vi "MQTT Packet - Send.vi"(0 "mqtt ref in":T1, 7 "packet data":u8[](array[numeric]), 9 "MessageType":T3, 11 "error in (no error)":errorcluster, 12 "Retain":bool, 13 "QoS":T2, 14 "DUP":bool) -> (3 "Debug":string, 4 "mqtt ref out":T1, 15 "error out":errorcluster)   [LabVIEW 2019, in "KoRE-MQTT.lvlib"]
doc: "Copyright (c) 2025 KoRElibs.com\nSPDX-License-Identifier: EUPL-1.2\n\nThis VI is licensed under the European Union Public License (EUPL) Version 1.2. You may use this VI unmodified in proprietary works. If you distribute a modified version of this file, the modified file must be released under the EUPL-1.2. Full license: https://joinup.ec.europa.eu/asset/eupl/eupl/1.2/"
uses:
  KoRE-MQTT.lvlib
  TypeDefs/MQTT Packet - Type.ctl
  Public/TypeDefs/MQTT QoS Level.ctl
  Public/TypeDefs/MQTT Client Session.ctl
  MQTT Data - Encode Varint.vi
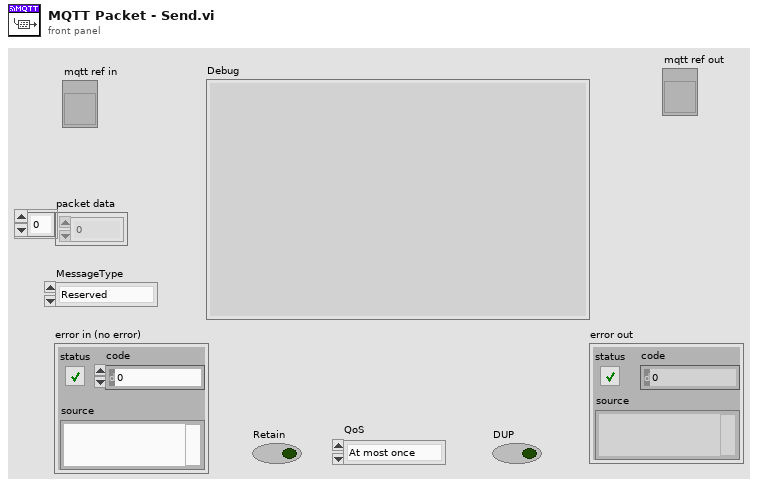
[diagram p1: front panel]
types:
  T1 = typedef "KoRE-MQTT.lvlib/MQTT Client Session.ctl" = refnum<vi>
  T2 = typedef "KoRE-MQTT.lvlib/MQTT QoS Level.ctl" = enum8{"At most once", "At least once", "Exactly once"}
  T3 = typedef "KoRE-MQTT.lvlib/MQTT Packet - Type.ctl" = enum32{"Reserved", "CONNECT", "CONNACK", "PUBLISH", "PUBACK", "PUBREC", "PUBREL", "PUBCOMP", "SUBSCRIBE", "SUBACK", "UNSUBSCRIBE", "UNSUBACK", "PINGREQ", "PINGRESP", "DISCONNECT", "AUTH"}
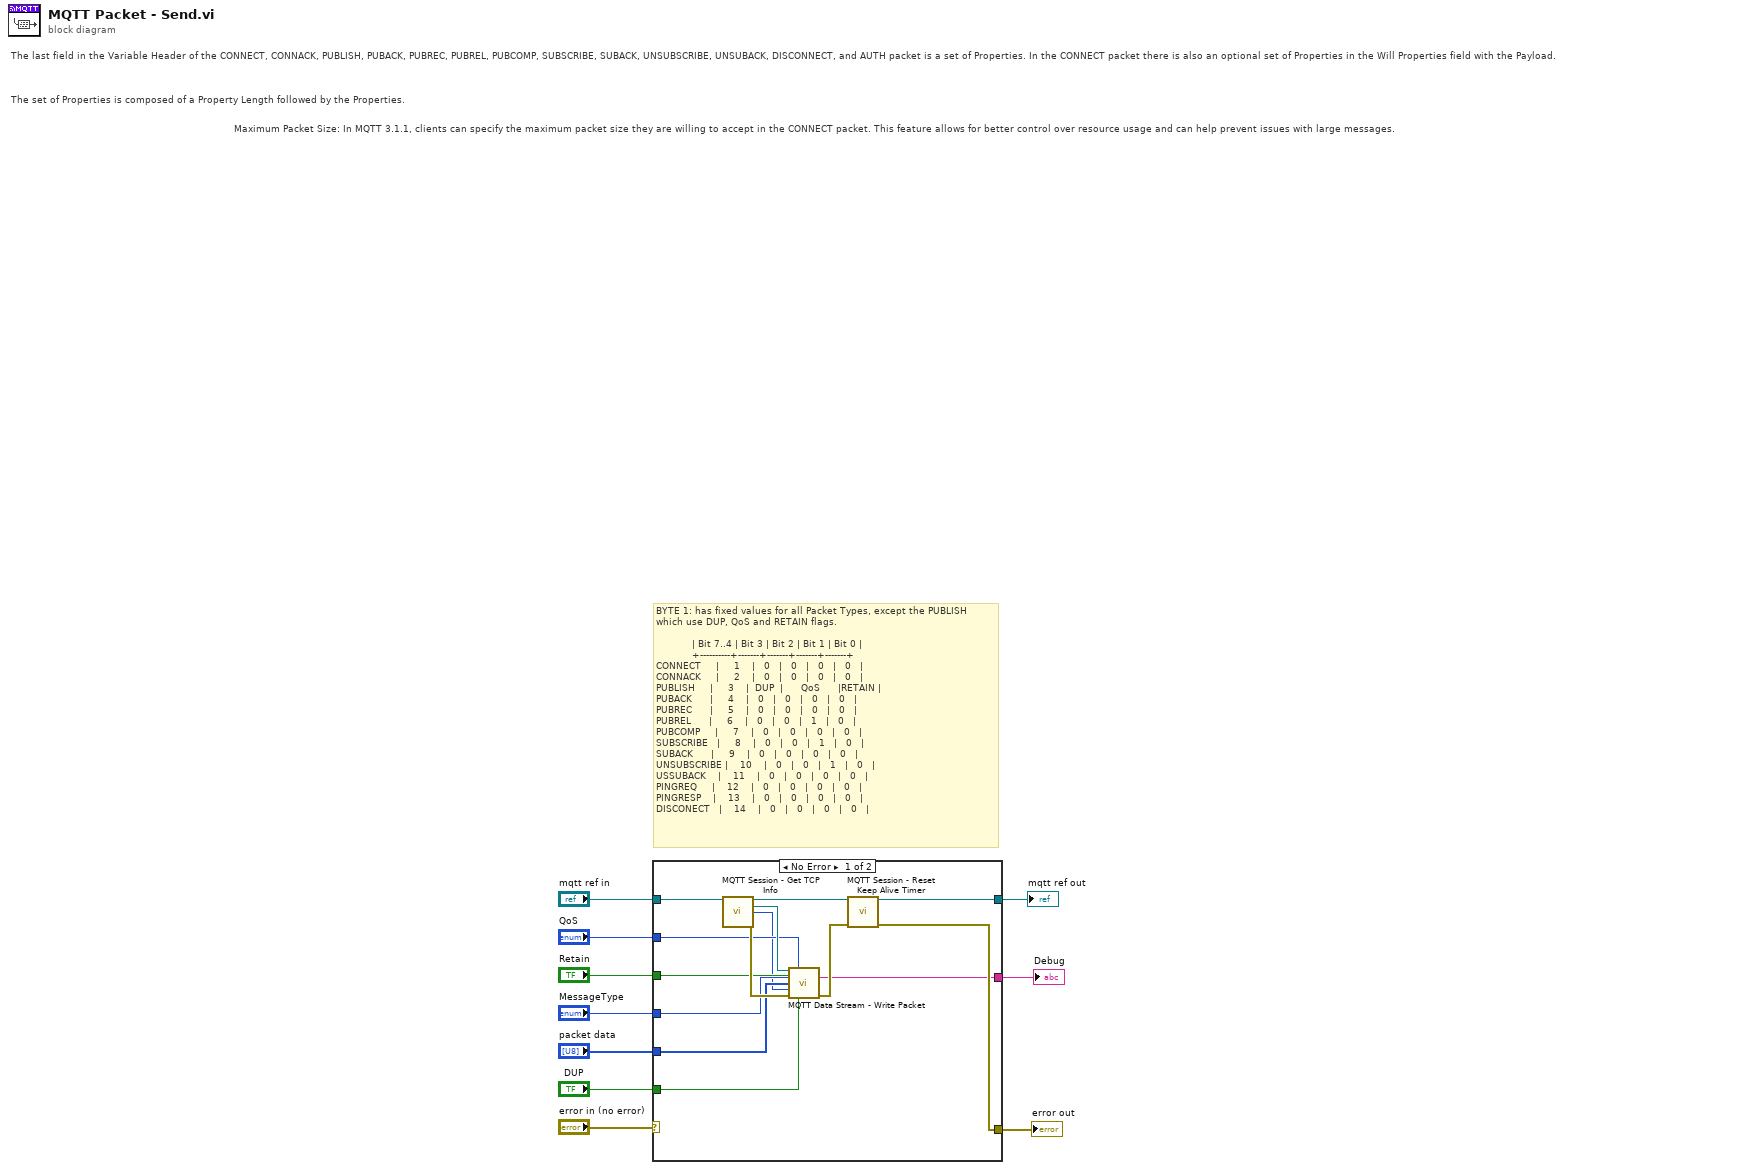
[diagram p0: block diagram]
diagram:
  # "BYTE 1: has fixed values for all Packet Types, except the PUBLISH which use DUP, QoS and RETAIN flags.\n\n            | Bit 7..4 | Bit 3 | Bit 2 | Bit 1 | Bit 0 |\n            +----------+-------+-------+-------+-------+\nCONNECT     |     1    |   0   |   0   |   0   |   0   |\nCONNACK     |     2    |   0   |   0   |   0   |   0   |\nPUBLISH     |     3    |  DUP  |      QoS      |RETAIN |\nPUBACK      |     4    |   0   |   0   |   0   |   0   |\nPUBREC      |     5    |   0   |   0   |   0   |   0   |\nPUBREL      |     6    |   0   |   0   |   1   |   0   |\nPUBCOMP     |     7    |   0   |   0   |   0   |   0   |\nSUBSCRIBE   |     8    |   0   |   0   |   1   |   0   |\nSUBACK      |     9    |   0   |   0   |   0   |   0   |\nUNSUBSCRIBE |    10    |   0   |   0   |   1   |   0   |\nUSSUBACK    |    11    |   0   |   0   |   0   |   0   |\nPINGREQ     |    12    |   0   |   0   |   0   |   0   |\nPINGRESP    |    13    |   0   |   0   |   0   |   0   |\nDISCONECT   |    14    |   0   |   0   |   0   |   0   |"
  # "Maximum Packet Size: In MQTT 3.1.1, clients can specify the maximum packet size they are willing to accept in the CONNECT packet. This feature allows for better control over resource usage and can help prevent issues with large messages."
  # "The last field in the Variable Header of the CONNECT, CONNACK, PUBLISH, PUBACK, PUBREC, PUBREL, PUBCOMP, SUBSCRIBE, SUBACK, UNSUBSCRIBE, UNSUBACK, DISCONNECT, and AUTH packet is a set of Properties. In the CONNECT packet there is also an optional set of Properties in the Will Properties field with the Payload.\n\n \n\nThe set of Properties is composed of a Property Length followed by the Properties."
  n1 = case shown="No Error" "error in (no error)" {
    selector: "error in (no error)" -> [_ w26]
    tunnel: "packet data" -> [w13 _]
    tunnel: "MessageType" -> [w15 _]
    tunnel: "QoS" -> [w17 _]
    tunnel: "DUP" -> [w14 _]
    tunnel: "Retain" -> [w16 _]
    tunnel: [w23 w26] -> w5
    tunnel: "mqtt ref in" -> [w19 w25]
    tunnel: [w24 w25] -> w2
    tunnel: [w11 _] -> w1
    frame No Error {
      n2 = call "MQTT Session - Get TCP Info.vi"("mqtt ref in"=w19) -> ("mqtt ref out"=w20:T1, "TCP ref"=w22:refnum<k5>, "TCP Timeout (ms)"=w12:i32, "error out"=w21:errorcluster)  [unwired: 10 in, 1 out]
      n3 = call "MQTT Data Stream - Write Packet.vi"("TCP Network Connection in"=w22, "QoS"=w17, "Retain"=w16, "MessageType"=w15, "packet data"=w13, "TCP Timeout"=w12, "error in (no error)"=w21, "DUP"=w14) -> ("DEBUG"=w11:string, "error out"=w18:errorcluster)  [unwired: 5 in, 1 out]
      n4 = call "MQTT Session - Reset Keep Alive Timer.vi"("MQTT_Q In in"=w20, "error in"=w18) -> ("MQTT_Q In out"=w24:T1, "error out"=w23:errorcluster)  [unwired: 12 in]
    }
    frame Error {
    }
  }
  "error out" <- w5
  "mqtt ref out" <- w2
  "Debug" <- w1
